vi "Regex Call Probe.vi"(0 "input string":string, 5 "regular expression":string, 11 "error in":errorcluster) -> (4 "whole match":string, 6 "matched substrings":string[](array[string]), 15 "error out":errorcluster)   [LabVIEW 2026]
doc: "Probe: Match Regular Expression through the XNode's Execute VI as a plain subVI call."
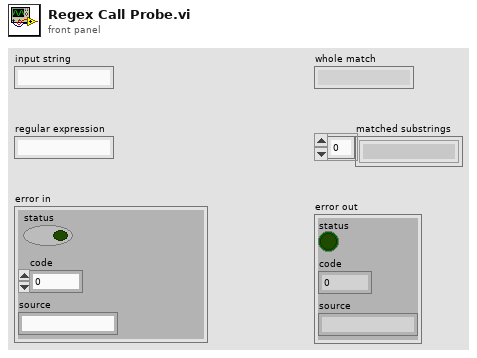
[diagram p1: front panel]
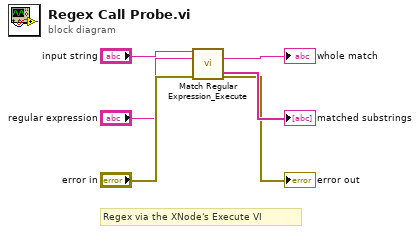
[diagram p0: block diagram]
diagram:
  # "Regex via the XNode's Execute VI"
  n1 = call "Match Regular Expression_Execute.vi"("input string"="input string", "regular expression"="regular expression", "error in (no error)"="error in") -> ("whole match"=→"whole match":string, "matched substrings"=→"matched substrings":string[], "error out"=→"error out":errorcluster)  [unwired: 7 in, 3 out]
